vi "Streaming Example.vi"() -> ()   [LabVIEW 2020]
uses:
  g_industrial_cam/Device Enumeration.ctl
  g_industrial_cam/Camera/Camera.lvclass/Camera.ctl
  g_industrial_cam/Buffer/Buffer.lvclass/Buffer.ctl
  g_industrial_cam/Camera/GetSetPixelFormat.vi
  g_industrial_cam/Buffer/Access Handle.vi
  g_industrial_cam/Buffer/Draw to Picture.vi
  g_industrial_cam/Buffer/Draw Mono8 to Picture.vi
  g_industrial_cam/Buffer/Draw Mono10 to Picture.vi
  g_industrial_cam/Buffer/Draw Mono12 to Picture.vi
  g_industrial_cam/Buffer/Draw Mono14 to Picture.vi
  g_industrial_cam/Buffer/Draw Mono16 to Picture.vi
  g_industrial_cam/Buffer/Draw Mono10p to Picture.vi
  g_industrial_cam/Buffer/Draw Mono12p to Picture.vi
  g_industrial_cam/Buffer/Draw Mono14p to Picture.vi
  g_industrial_cam/Buffer/Draw RGB8 to Picture.vi
  g_industrial_cam/Buffer/Draw BGR8 to Picture.vi
  g_industrial_cam/Buffer/Get Image Size.vi
  g_industrial_cam/Buffer/Scale Picture to Centre Image.vi
  g_industrial_cam/Buffer/DrawToPictureCore.vi
  g_industrial_cam/Buffer/GetBufferImageDimensions.vi
  g_industrial_cam/Camera/Check Not Disconnected.vi
  <vilib>/Utility/error.llb/Error Cluster From Error Code.vi
  g_industrial_cam/Camera/Destroy Stream Events.vi
  g_industrial_cam/Camera/Check Stream OK.vi
  g_industrial_cam/Buffer/Buffer.lvclass
  g_industrial_cam/Camera/Camera.lvclass
panel:
  out "Iterations":i32
  out "Pixel Formats":string[](array[string])
  out "Frame-Error Count":u64
  out "Frame Count (inc Errors)":u64
  out "Timeout":bool
  out "Devices":T1[](array[typedef])
  out "Picture":picture
  in  "stop":bool
  out "error out":errorcluster
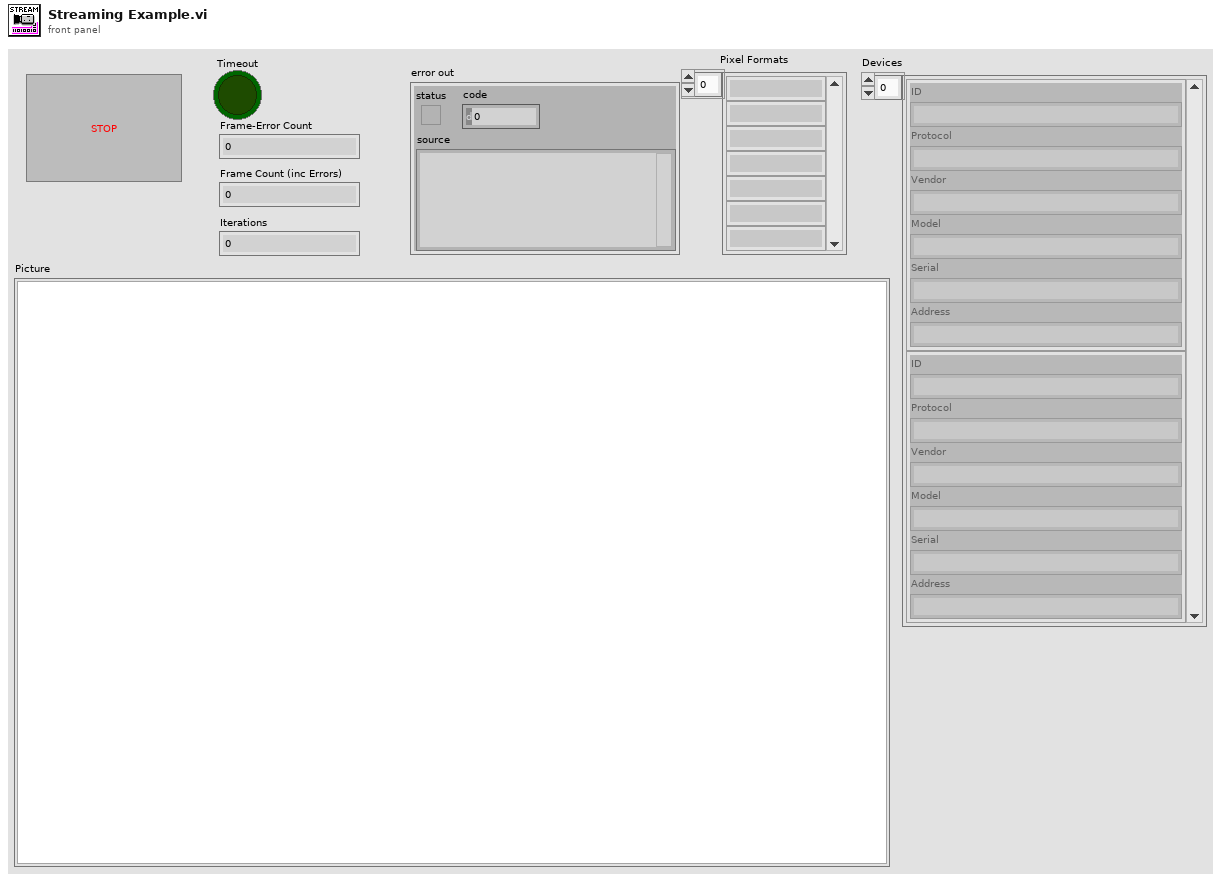
[diagram p1: front panel]
types:
  T1 = typedef "Device Enumeration.ctl" = cluster{"ID":string, "Protocol":string, "Vendor":string, "Model":string, "Serial":string, "Address":string}
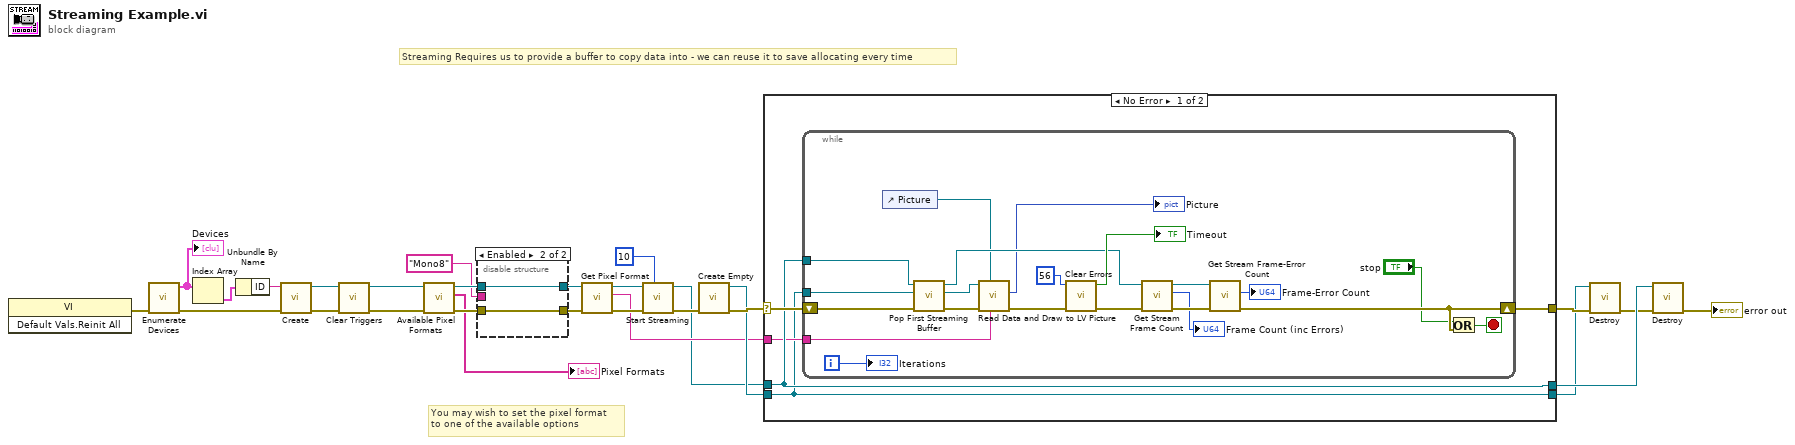
[diagram p0: block diagram]
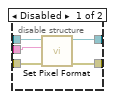
[diagram p2: hidden frame]
diagram:
  # "You may wish to set the pixel format\nto one of the available options"
  # "Streaming Requires us to provide a buffer to copy data into - we can reuse it to save allocating every time"
  n1 = invoke class="VI" method="Default Vals.Reinit All"() -> (error out=w7:errorcluster)  [unwired: 3 in, 2 out]
  n2 = call "Enumerate Devices.vi"("error in (no error)"=w7) -> ("error out"=w26:errorcluster, "Devices"=w28:T1[])  [unwired: 9 in]
  "Devices" <- w28
  n3 = Index Array(array=w28) -> (element=w27:T1)  [unwired: 1 in]
  n4 = Unbundle By Name(w27) -> ("ID"=w25:string)
  n5 = call "Create.vi"("error in (no error)"=w26, "Identifier (ID, IP etc)"=w25) -> ("error out"=w5:errorcluster, "Camera"=w6:refnum<class "Camera.lvclass">)  [unwired: 8 in]
  n6 = call "Clear Triggers.vi"("error in (no error)"=w5, "Camera in"=w6) -> ("error out"=w4:errorcluster, "Camera"=w3:refnum<class "Camera.lvclass">)  [unwired: 8 in]
  n7 = call "Available Pixel Formats.vi"("error in (no error)"=w4, "Camera in"=w3) -> ("error out"=w13:errorcluster, "Pixel Formats"=→"Pixel Formats":string[], "Camera"=w10:refnum<class "Camera.lvclass">)  [unwired: 7 in]
  n8 = disable-structure shown="Enabled" {
    disable-tunnel: w13 -> [w33 w34]
    disable-tunnel: [w32 w34] -> w11
    disable-tunnel: w10 -> [w31 w35]
    disable-tunnel: [w30 w35] -> w9
    disable-tunnel: "Mono8" ("Pixel Format") -> [w29 _]
    frame Disabled {
      n9 = call "Set Pixel Format.vi"("error in (no error)"=w33, "Pixel Format"=w29, "Camera in"=w31) -> ("error out"=w32:errorcluster, "Camera"=w30:refnum<class "Camera.lvclass">)  [unwired: 7 in]
    }
    frame Enabled {
    }
  }
  n10 = call "Get Pixel Format.vi"("error in (no error)"=w11, "Camera in"=w9) -> ("error out"=w19:errorcluster, "Pixel Format"=w17:string, "Camera"=w18:refnum<class "Camera.lvclass">)  [unwired: 7 in]
  n11 = call "Start Streaming.vi"("Additional Buffers (Default: 3)"=u16 10, "error in (no error)"=w19, "Camera in"=w18) -> ("error out"=w24:errorcluster, "Camera"=w2:refnum<class "Camera.lvclass">)  [unwired: 7 in]
  n12 = call "Create Empty.vi"("error in (no error)"=w24) -> ("error out"=w23:errorcluster, "Empty Buffer"=w22:refnum<class "Buffer.lvclass">)  [unwired: 9 in]
  n13 = case shown="No Error" w23 {
    selector: w23 -> [w40 w63]
    tunnel: w2 -> [w38 w64]
    tunnel: [w39 w63] -> w16
    tunnel: [w38 w64] -> w21
    tunnel: w22 -> [w36 w62]
    tunnel: w17 -> [w37 _]
    tunnel: [w36 w62] -> w14
    frame No Error {
      n14 = while {
        shift-right: [w59] -> w39
        shift-left: w40 -> [w58]
        tunnel: w38 -> [w61]
        tunnel: w37 -> [w57]
        tunnel: w36 -> [w56]
        i -> [w41]
        stop <- w60 stop-if-true
        n15 = control-ref of="Picture"() -> (w43:refnum<vi>)
        n16 = call "Pop First Streaming Buffer.vi"("error in (no error)"=w58, "Buffer in"=w56, "Camera in"=w61) -> ("error out"=w48:errorcluster, "Buffer"=w46:refnum<class "Buffer.lvclass">, "Camera"=w45:refnum<class "Camera.lvclass">)  [unwired: 6 in]
        n17 = call "Read Data and Draw to LV Picture.vi"("Pixel Format"=w57, "Picture Ref"=w43, "error in (no error)"=w48, "Buffer in"=w46) -> ("error out"=w47:errorcluster, "Picture"=→"Picture":picture)  [unwired: 5 in, 1 out]
        n18 = call <vilib>:"Clear Errors.vi"("error in (no error)"=w47, "specific error code to clear (0: all)"=56) -> ("error out"=w55:errorcluster, "specific error cleared?"=→"Timeout":bool)  [unwired: 4 in]
        n19 = call "Get Stream Frame Count.vi"("error in (no error)"=w55, "Camera in"=w45) -> ("error out"=w52:errorcluster, "Frame Count (inc Errors)"=→"Frame Count (inc Errors)":u64, "Camera"=w51:refnum<class "Camera.lvclass">)  [unwired: 7 in]
        n20 = call "Get Stream Frame-Error Count.vi"("error in (no error)"=w52, "Camera in"=w51) -> ("error out"=w59:errorcluster, "Frame-Error Count"=→"Frame-Error Count":u64)  [unwired: 7 in, 1 out]
        n21 = Or(x="stop", y=w59) -> (x .or. y?=w60:bool)
        "Iterations" <- w41
      }
    }
    frame Error {
    }
  }
  n22 = call "Destroy.vi"("error in (no error)"=w16, "Buffer in"=w14) -> ("error out"=w15:errorcluster)  [unwired: 9 in]
  n23 = call "Destroy.vi"("error in (no error)"=w15, "Camera in"=w21) -> ("error out"=→"error out":errorcluster)  [unwired: 9 in]
